vi "Assert Pass.vi"(8 "error in (no error)":errorcluster, 10 "Mock":refnum<class "LMock Mock.lvclass">, 11 "Tolerant Numeric Comparator Test In":refnum<class "Tolerant Numeric Comparator Test.lvclass">) -> (0 "error out":errorcluster, 3 "Tolerant Numeric Comparator Test Out":refnum<class "Tolerant Numeric Comparator Test.lvclass">)   [LabVIEW 2020, in "Tolerant Numeric Comparator Test.lvclass"]
uses:
  Tolerant Numeric Comparator Test.lvclass
  C:/Program Files (x86)/National Instruments/LabVIEW 2020/vi.lib/Astemes/LUnit/Test Case.lvclass
  source/Framework/Mock/LMock Mock.lvclass
  <vilib>/Astemes/LUnit/Test Case.lvclass/Test Case.ctl
  <vilib>/Astemes/LUnit/Append Fail Result.vi
  <vilib>/Astemes/LUnit/Append Pass Result.vi
  <vilib>/Astemes/LUnit/Test Case.lvclass
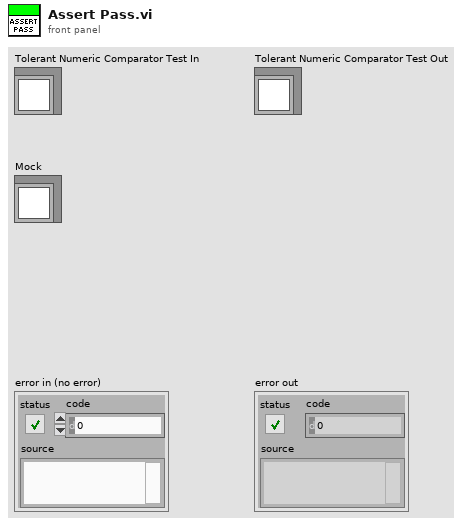
[diagram p1: front panel]
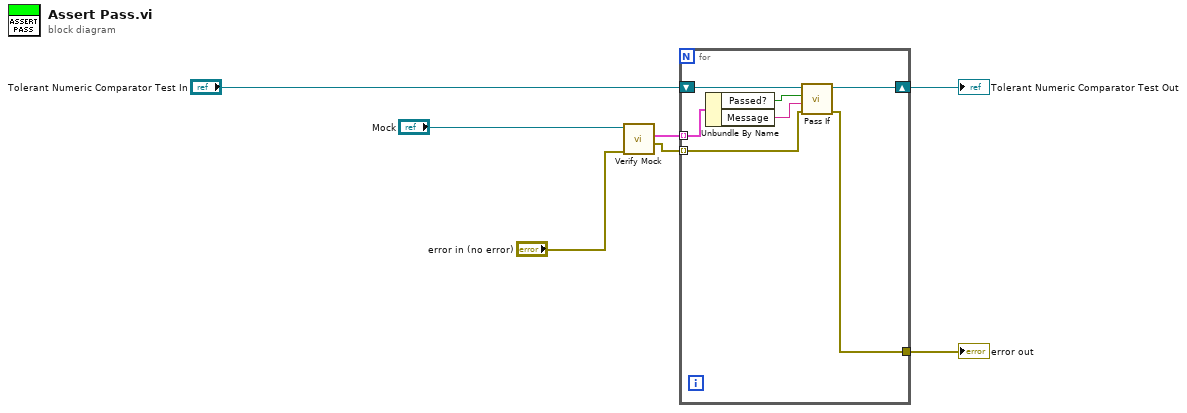
[diagram p0: block diagram]
diagram:
  n1 = call-dynamic "Verify Mock.vi"("error in (no error)"="error in (no error)", "Mock In"="Mock") -> ("Errors"=w4:errorcluster[], "Results"=w5:cluster{"Passed?":bool, "Message":string}[])  [unwired: 7 in, 1 out]
  n2 = for {
    tunnel: [w13] -> w2
    tunnel: w4 -> [w12] mode=indexing
    tunnel: w5 -> [w10] mode=indexing
    shift-right: [w14] -> w1
    shift-left: "Tolerant Numeric Comparator Test In" -> [w11]
    n3 = Unbundle By Name(w10) -> ("Passed?"=w9:bool, "Message"=w8:string)
    n4 = call <vilib>:"Pass If.vi"("error in (no error)"=w12, "Message"=w8, "Pass?"=w9, "LUnit Test Case In"=w11) -> ("error out"=w13:errorcluster, "LUnit Test Case Out"=w14:refnum<class "Tolerant Numeric Comparator Test.lvclass">)  [unwired: 6 in]
  }
  "error out" <- w2
  "Tolerant Numeric Comparator Test Out" <- w1
